vi "VIH HelpGen - HTML - Escape Characters in URL.vi"(9 "Escape mailto Reserved chars (F)":bool, 10 "Escape HTML Reserved chars (T)":bool=TRUE, 11 "string":string) -> (3 "URL string":string)   [LabVIEW 2014]
doc: "::: VI Helpeks :::\nCopyright (c) 2000-2026 Konstantin Shifershteyn. All rights reserved."
panel:
  # "VI Helpeks\nCopyright (c) 2012-2026 Konstantin Shifershteyn"
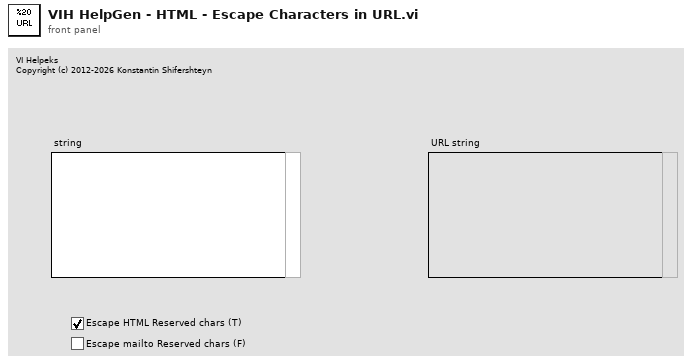
[diagram p1: front panel]
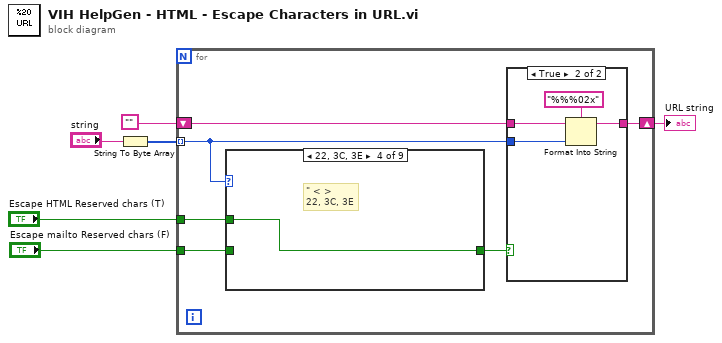
[diagram p0: block diagram]
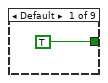
[diagram p2: hidden frame]
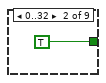
[diagram p3: hidden frame]
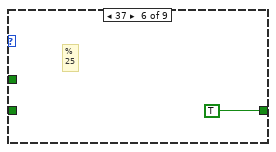
[diagram p6: hidden frame]
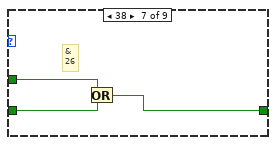
[diagram p7: hidden frame]
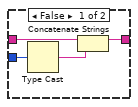
[diagram p10: hidden frame]
diagram:
  n1 = String To Byte Array(string="string") -> (unsigned byte array=w5:u8[])
  n2 = for {
    tunnel: w5 -> [w10] mode=indexing
    shift-right: [w11] -> w3
    shift-left: "" -> [w12]
    tunnel: "Escape HTML Reserved chars (T)" -> [w8]
    tunnel: "Escape mailto Reserved chars (F)" -> [w7]
    n3 = case shown="22, 3C, 3E" w10 {
      tunnel: [TRUE TRUE _ w15 _ TRUE w17 _ w20] -> w9
      tunnel: w8 -> [_ _ _ w15 _ _ w19 _ _]
      tunnel: w7 -> [_ _ _ _ _ _ w18 _ w20]
      frame Default {
      }
      frame 0..32 {
      }
      frame 33, 36, 40..44, 59 {
        # "! $ ' ( ) * + , ; =\n21, 24, 28, 29, 2A, 2B, 2C, 3B"
      }
      frame 34, 60, 62 {
        # "\" < >\n22, 3C, 3E"
      }
      frame 35, 47, 58, 64, 91, 93 {
        # "# / : @ [ ]\n23, 2F, 3A, 40, 5B, 5D"
      }
      frame 37 {
        # "%\n25"
      }
      frame 38 {
        # "&\n26"
        n4 = Or(x=w19, y=w18) -> (x .or. y?=w17:bool)
      }
      frame 45, 46, 48..57, 65..90, 95, 97..122, 126 {
        # "- . 0-9 A-Z _ a-z ~\n2D, 2E, 30..39, 41 .. 5A, 5F, 61..7A, 7E"
      }
      frame 61, 63 {
        # "= ?\n3D, 3F"
      }
    }
    n5 = case shown="True" w9 {
      tunnel: w12 -> [w24 w27]
      tunnel: [w23 w26] -> w11
      tunnel: w10 -> [w21 w25]
      frame False {
        n6 = Type Cast(x=w21) -> (*(type *) &x=w22:string)  [unwired: 1 in]
        n7 = Concatenate Strings(w24, w22) -> (w23:string)
      }
      frame True {
        n8 = Format Into String(format string="%%%02x" ("Format String"), initial string=w27, w25) -> (resulting string=w26:string)  [unwired: 1 in, 1 out]
      }
    }
  }
  "URL string" <- w3
